vi "AddAuth.vi"(8 "error in (no error)":errorcluster, 10 "ApiKey":string, 11 "client handle in":T1) -> (0 "error out":errorcluster, 3 "client handle out":T1)   [LabVIEW 2017]
uses:
  <vilib>/httpClient/ClientHandle.ctl
  <vilib>/httpClient/LabVIEWHTTPClient.lvlib
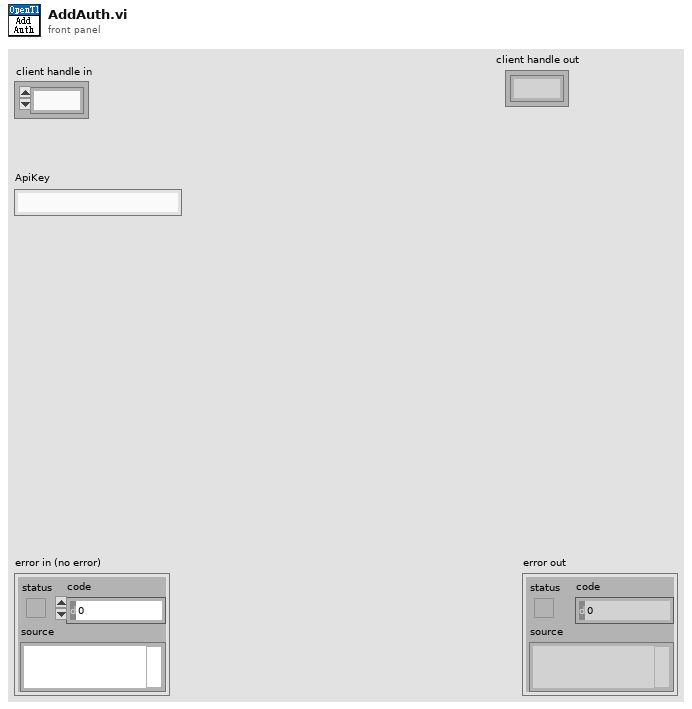
[diagram p1: front panel]
types:
  T1 = typedef "LabVIEWHTTPClient.lvlib/ClientHandle.ctl" = refnum<k1>
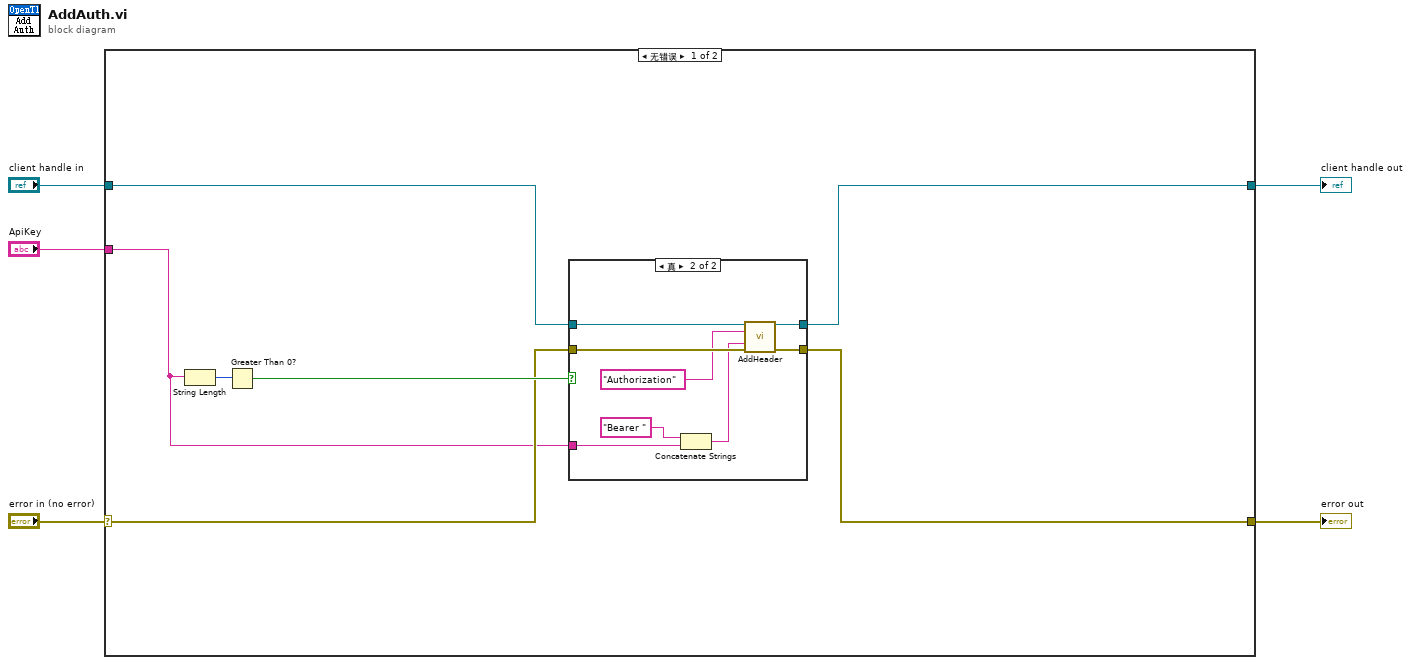
[diagram p0: block diagram]
diagram:
  n1 = case shown="无错误" "error in (no error)" {
    selector: "error in (no error)" -> [w9 w24]
    tunnel: [w7 w24] -> w4
    tunnel: "client handle in" -> [w12 w23]
    tunnel: "ApiKey" -> [w8 _]
    tunnel: [w6 w23] -> w1
    frame No Error {
      n2 = String Length(string=w8) -> (length=w11:i32)
      n3 = Greater Than 0?(x=w11) -> (x > 0?=w10:bool)
      n4 = case shown="真" w10 {
        tunnel: w12 -> [w14 w22]
        tunnel: [w14 w21] -> w6
        tunnel: w9 -> [w13 w20]
        tunnel: [w13 w19] -> w7
        tunnel: w8 -> [_ w16]
        frame False {
        }
        frame True {
          n5 = Concatenate Strings("Bearer " ("url"), w16) -> (w18:string)
          n6 = call <vilib>:"AddHeader.vi"("client handle"=w22, "header"="Authorization" ("url"), "value"=w18, "error in (no error)"=w20) -> ("client handle out"=w21:T1, "error out"=w19:errorcluster)  [unwired: 10 in]
        }
      }
    }
    frame Error {
    }
  }
  "error out" <- w4
  "client handle out" <- w1
